vi "pi_control.vi"() -> ()   [LabVIEW 2020]
uses:
  <vilib>/Platform/TimedLoop/XDataNode/timing_clust.ctl
  <vilib>/Platform/TimedLoop/XDataNode/nitl_modes.ctl
  <vilib>/Platform/TimedLoop/XDataNode/wakeup.ctl
  <vilib>/Model Interface Toolkit/Model Interface Toolkit.lvclass/Model Interface Toolkit.ctl
  <vilib>/Model Interface Toolkit/Model Update.vi
  <vilib>/Model Interface Toolkit/Tick Model.vi
  <vilib>/Model Interface Toolkit/Probe Signals.vi
  <vilib>/Model Interface Toolkit/Multirate/Dispatch Model Tasks.vi
  <vilib>/Model Interface Toolkit/Call Model Start Routine.vi
  <vilib>/Model Interface Toolkit/Handle Error.vi
  <vilib>/Model Interface Toolkit/Multirate/Wait on Tasks.vi
  <vilib>/Model Interface Toolkit/Get Inport Paths.vi
  <vilib>/Model Interface Toolkit/Get Outport Paths.vi
  <vilib>/Model Interface Toolkit/Check Error.vi
  <vilib>/Model Interface Toolkit/Generate Error Cluster.vi
  <vilib>/Platform/TimedLoop/scheduler/LVUserAPI/Fire Software-Triggered Timing Source.vi
  <vilib>/Platform/TimedLoop/XDataNode/XDataNode.xnode
  <vilib>/Model Interface Toolkit/Model Interface Toolkit.lvclass
  <vilib>/Platform/TimedLoop/XDataNode/XDNodeRunTimeDep.lvlib
panel:
  in  "选项卡控件":enum32{"参数配置", "控制器及车辆状态评估"}(tab)
  out "Inports":string[](array[string])
  out "Outports":string[](array[string])
  in  "Model Path":path=path "C:/ni-rt/NIVeriStand2010/Models/TSMC_V2.dll"
  in  "数据储存路径":path=path "C:/ni-rt/startup/data/test5.tdms"
  out "controler output data":dbl[](array[numeric])
  out "CarSim Output Data":dbl[](array[numeric]) format="%.2f"
  out "Time Step":dbl=0.001 format="%.4f"
  out "Current Time":dbl format="%.2f"
  out "Start Time":dbl format="%.2f"
  out "Stop Time":dbl=0.001 format="%.4f"
  out "Overrun":i32
  out "x*y":dbl
  out "相平面图":cluster{"X":dbl, "Y":dbl}[](graph)
  out "瞬态误差":cluster{"下界":dbl, "误差":dbl, "上界":dbl}(graph)
  out "波形图表":T1(graph)
  in  "stop":bool
  # "Simulation"
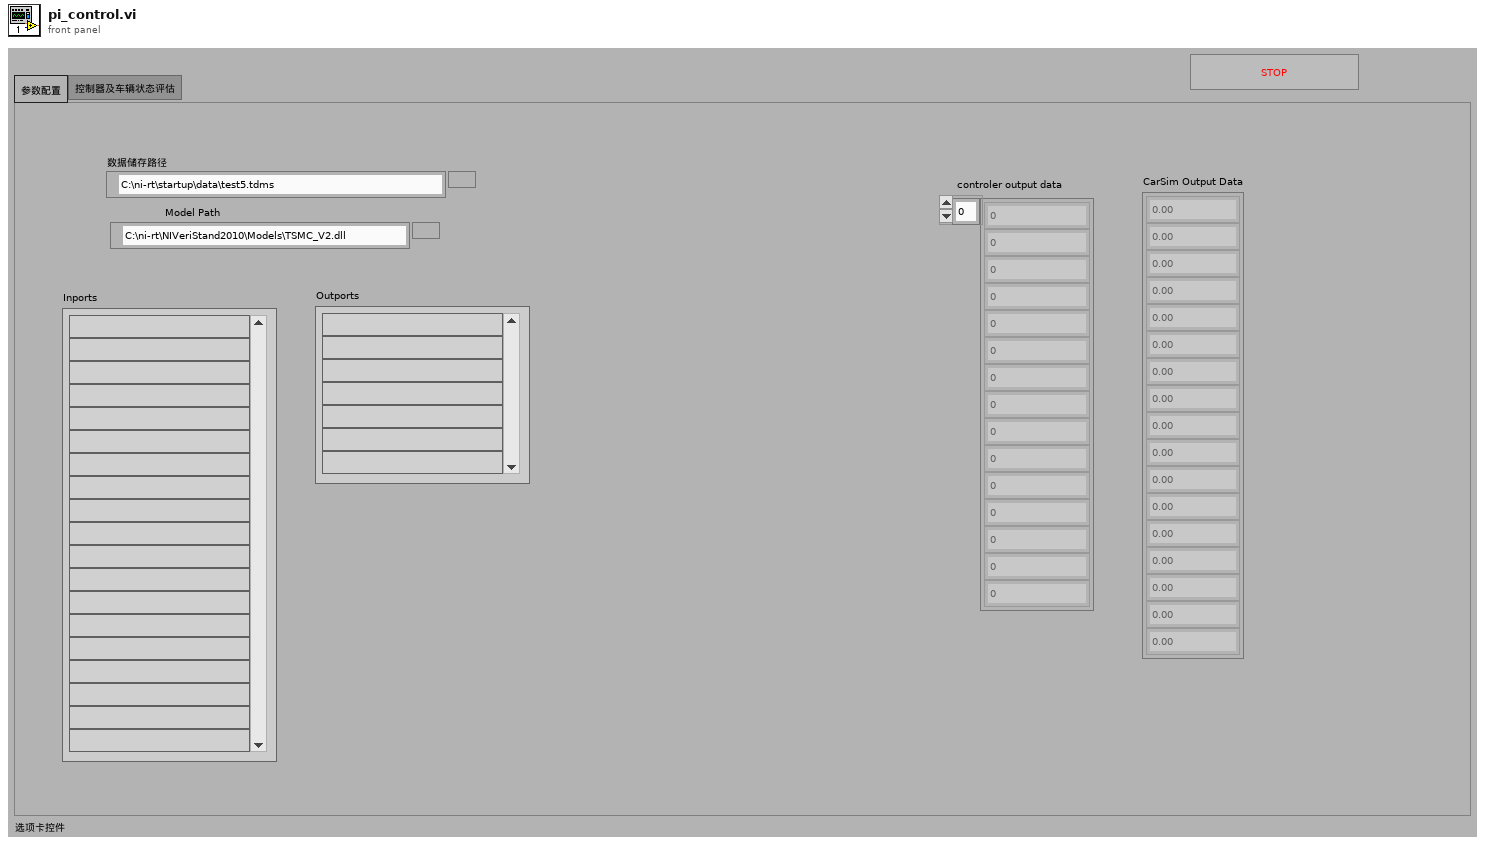
[diagram p1: front panel]
types:
  T1 = cluster{"[0]":dbl, "[1]":dbl, "[2]":dbl, "[3]":dbl, "[4]":dbl}
  T2 = enum16{"open", "open or create", "create or replace", "create", "open (read-only)"}
  T3 = typedef "XDNodeRunTimeDep.lvlib/timing_clust.ctl" = cluster{"Expected End [f-1]":u64, "Actual End [f-1]":u64, "Finished Late? [f-1]":bool, "Expected End [i-1]":u64, "Actual End [i-1]":u64, "Finished Late? [i-1]":bool, "Expected Start [i]":u64, "Actual Start [i]":u64, "Expected Start [f]":u64, "Actual Start [f]":u64, "Source Name":string, "Structure Name":string, "Period":i64, "Deadline":i64, "Offset":i64, "Start":i64, "Priority":i32, "Timeout":i32, "Mode":T4, "Wakeup Reason":T5, "Error":errorcluster, "Source Type":string, "Secondary Source Type":string, "Global End Time":u64, "Global Start Time":u64, "Frame Duration":u64, "Iteration Duration":u64, "Assigned CPU":i32, "I/O Scan Engine Mode":u32}
  T4 = typedef "XDNodeRunTimeDep.lvlib/nitl_modes.ctl" = enum32{"No Change", "Process missed periods, maintain original phase", "Discard missed periods, maintain original phase", "Process missed periods, ignore original phase", "Discard missed periods, ignore original phase"}
  T5 = typedef "XDNodeRunTimeDep.lvlib/wakeup.ctl" = enum32{"Normal", "Aborted", "Asynchronous wakeup", "Timing source error", "Timed loop error", "Timeout"}
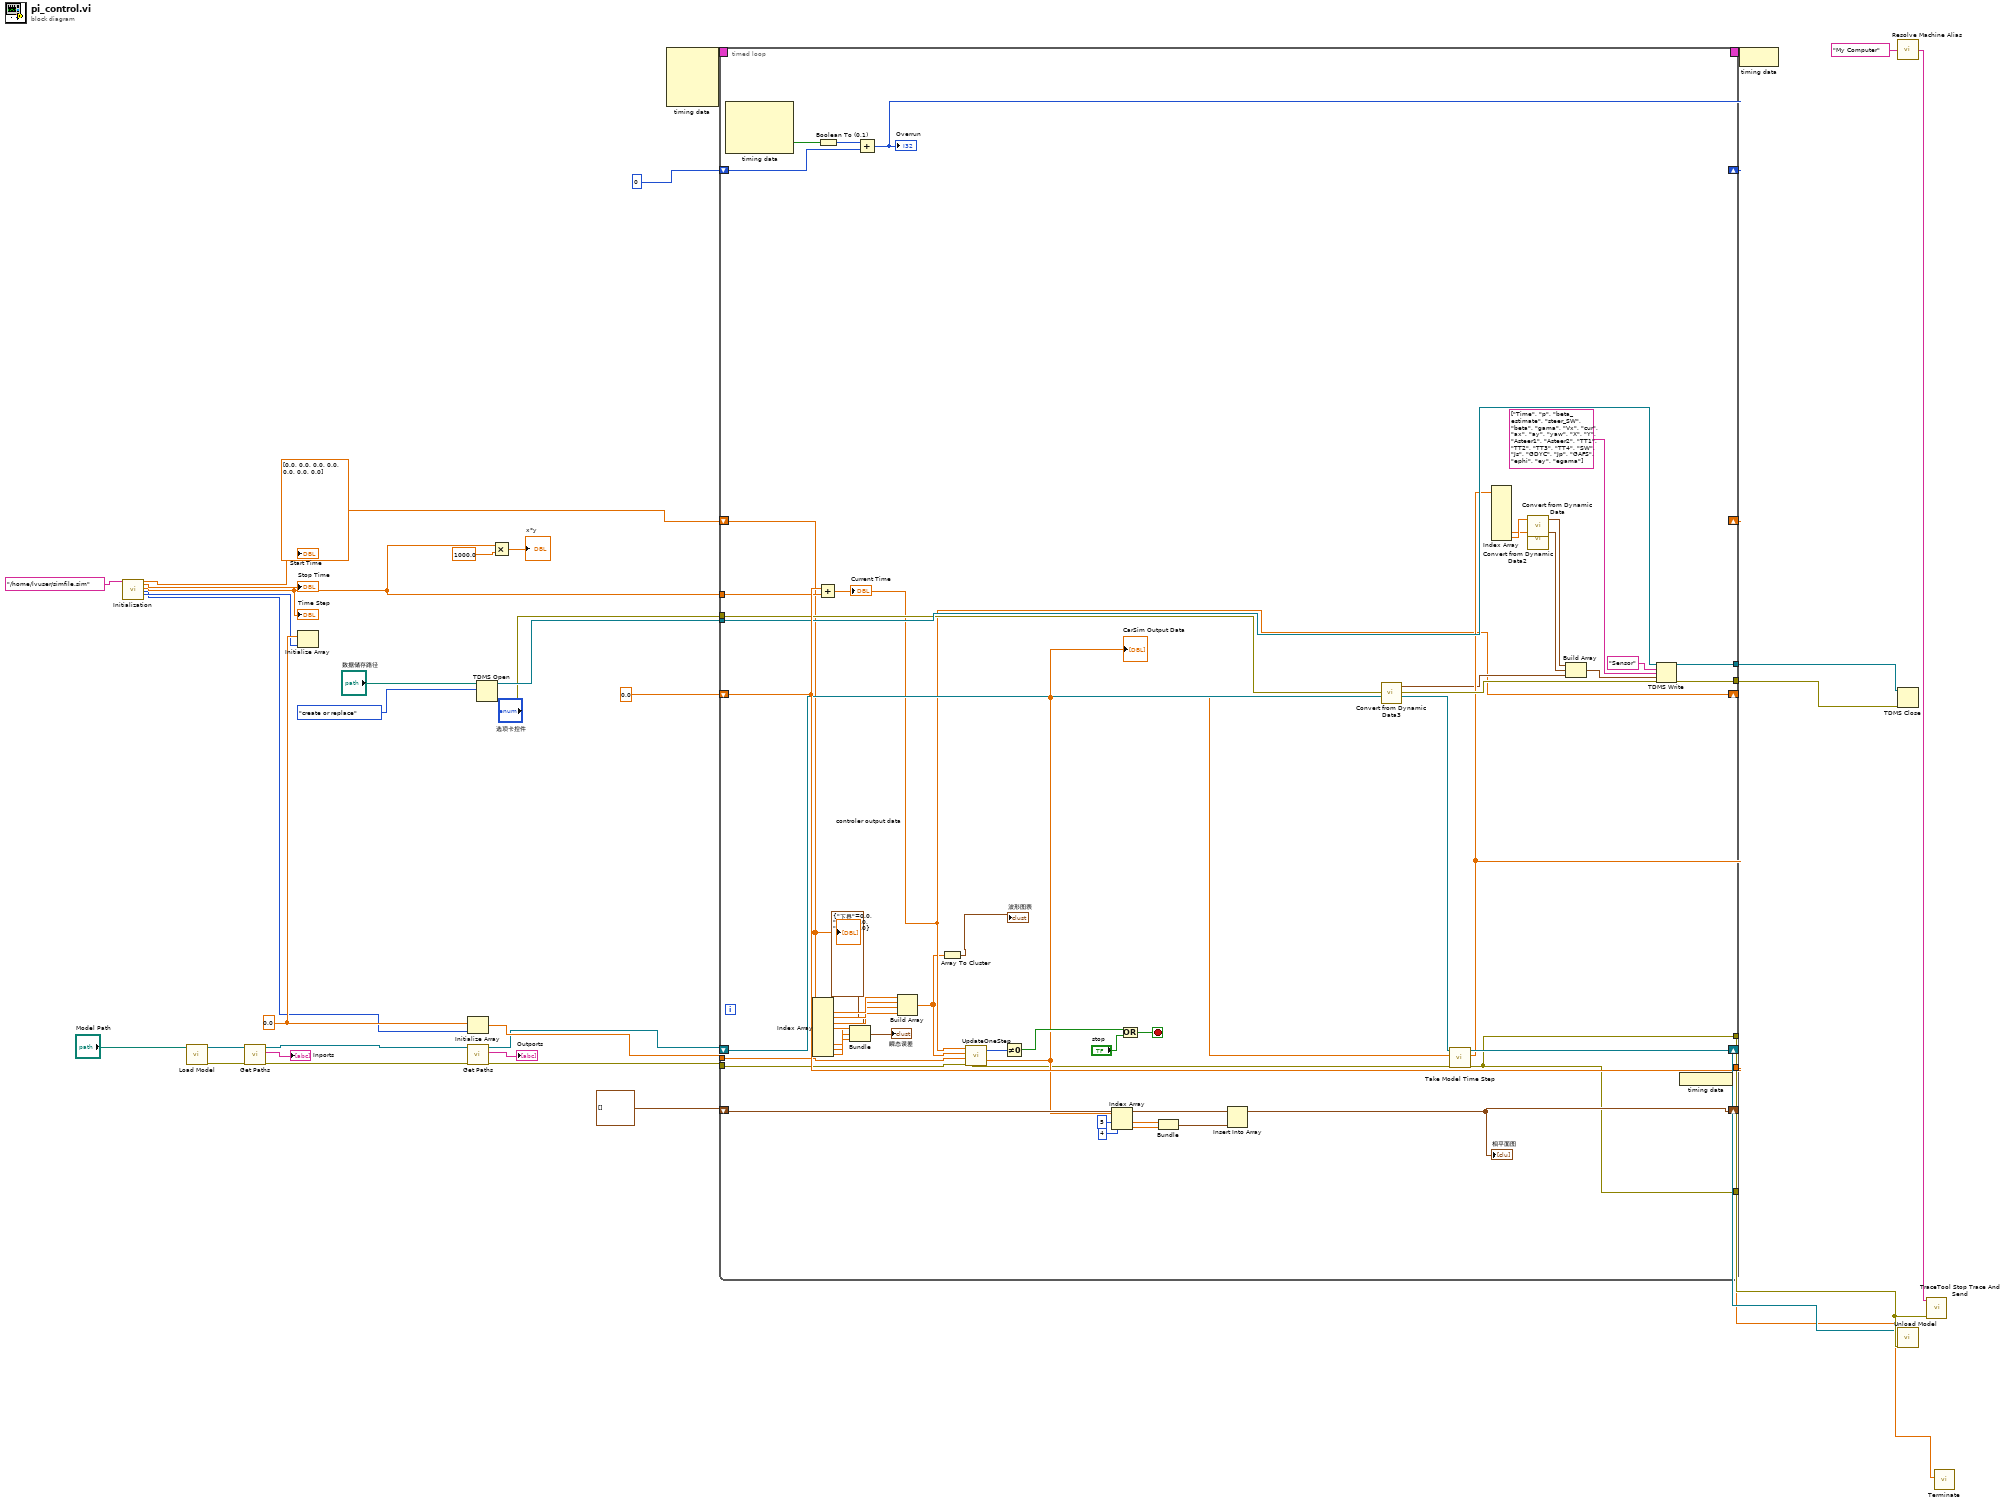
[diagram p0: block diagram]
diagram:
  w34 = 0.0
  n1 = call "Initialization.vi"("Simfile"="/home/lvuser/simfile.sim") -> ("Start Time"=→"Start Time":dbl, "Stop Time"=→"Stop Time":dbl, "Time Step"=w4:dbl, "Number Input"=w3:i16, "Number Output"=w2:i16)  [unwired: 13 in, 1 out]
  "Time Step" <- w4
  n2 = call <vilib>:"Load Model.vi"("Model Path"="Model Path") -> ("error out"=w22:errorcluster, "Model out"=w23:refnum<class "Model Interface Toolkit.lvclass">)  [unwired: 9 in]
  n3 = call-poly <vilib>:"Get Paths.vi"("error in (no error)"=w22, "Model in"=w23) -> ("error out"=w27:errorcluster, "Inport Paths"=→"Inports":string[], "Model out"=w26:refnum<class "Model Interface Toolkit.lvclass">)  [unwired: 7 in]
  n4 = Initialize Array ("初始化数组")(w34, w3) -> ()  [unwired: 1 out]
  n5 = Initialize Array ("初始化数组")(w34, w2) -> (w33:dbl[])
  n6 = call-poly <vilib>:"Get Paths.vi"("error in (no error)"=w27, "Model in"=w26) -> ("error out"=w20:errorcluster, "Outport Paths"=→"Outports":string[], "Model out"=w21:refnum<class "Model Interface Toolkit.lvclass">)  [unwired: 7 in]
  n7 = TDMS Open ("TDMS打开")(10:T2."create or replace" ("operation (0:open)"), 11:"数据储存路径") -> (0:w11:errorcluster, 3:w12:refnum<k34>)  [unwired: 5 in]
  n8 = Multiply ("乘")(x=w4, y=1000.0) -> (x*y=→"x*y":dbl)
  n9 = node-c288() -> (w36:T3)  [unwired: 4 in]
  n10 = timed-loop "定时循环" {
    timing: w36 -> [_]
    timing-out: [_] -> w35
    tunnel: w33 -> [w41]
    tunnel: w4 -> [w82]
    shift-right: [w43] -> _
    shift-left: 0.0 -> [w83]
    tunnel: [w83] -> w7
    shift-right: [w79] -> _
    shift-left: 0 -> [w80]
    tunnel: [w44] -> w19
    tunnel: w20 -> [w40]
    shift-right: [w67] -> _
    shift-left: dbl[] [0.0, 0.0, 0.0, 0.0, 0.0, 0.0, 0.0] ("Outport Array out") -> [w66]
    shift-right: [w76] -> w16
    shift-left: w21 -> [w77]
    tunnel: w12 -> [w75]
    tunnel: w11 -> [w74]
    tunnel: [w71] -> w10
    tunnel: [w70] -> w9
    shift-right: [w53] -> _
    shift-left: cluster{dbl, dbl}[] [] -> [w57]
    tunnel: [w44] -> _
    stop <- w85 stop-if-true
    n11 = node-c288() -> (w78:bool)  [unwired: 1 in, 3 out]
    n12 = Index Array(array=w66) -> (element #1=w61:dbl, element #2=w60:dbl, element #3=w59:dbl, element #4=w58:dbl, element #7=w45:dbl, element #8=w46:dbl, element #9=w47:dbl)  [unwired: 9 in, 2 out]
    n13 = Boolean To (0,1) ("布尔值至(0,1)转换")(Boolean=w78) -> (0, 1=w81:i16)
    n14 = Add ("加")(x=w83, y=w82) -> (x+y=w43:dbl)
    "Current Time" <- w43
    n15 = Bundle(cluster=cluster{"下界":dbl, "误差":dbl, "上界":dbl} {"下界"=0.0, "误差"=0.0, "上界"=0.0} ("簇"), "下界"=w45, "误差"=w46, "上界"=w47) -> (→"瞬态误差":cluster{"下界":dbl, "误差":dbl, "上界":dbl})
    n16 = Add ("加")(x=w81, y=w80) -> (x+y=w79:i32)
    "Overrun" <- w79
    n17 = Build Array ("创建数组")(w61, w60, w59, w58) -> (w42:dbl[])
    n18 = Array To Cluster ("数组至簇转换")(array=w42) -> (cluster=→"波形图表":T1)
    n19 = call "UpdateOneStep.vi"("error in (no error)"=w40, "init output"=w41, "input data"=w42, "time"=w43) -> ("error out"=w37:errorcluster, "output data"=w38:dbl[], "Func Return"=w39:i16)  [unwired: 5 in]
    "CarSim Output Data" <- w38
    n20 = Not Equal To 0? ("不等于0？")(x=w39) -> (x != 0?=w86:bool)
    n21 = Index Array(array=w38, index #1=5 ("索引"), index #2=4 ("索引")) -> (element #1=w55:dbl, element #2=w54:dbl)
    n22 = Or ("或")(x=w86, y="stop") -> (x .or. y?=w85:bool)
    n23 = Bundle(w55, w54) -> (w56:cluster{dbl, dbl})  [unwired: 1 in]
    n24 = Insert Into Array(array=w57, new element=w56) -> (w53:cluster{dbl, dbl}[])  [unwired: 1 in]
    "相平面图" <- w53
    n25 = call "Convert from Dynamic Data3"() -> ("Waveform"=w62:waveform(dbl))  [unwired: 4 in]
    n26 = call <vilib>:"Take Model Time Step.vi"("error in (no error)"=w37, "Inport Array"=w38, "Model in"=w77) -> ("error out"=w44:errorcluster, "Outport Array out"=w67:dbl[], "Model out"=w76:refnum<class "Model Interface Toolkit.lvclass">)  [unwired: 6 in]
    n27 = Index Array ("索引数组")(array=w67) -> (element #7=w63:dbl, element #8=w65:dbl)  [unwired: 8 in, 6 out]
    n28 = call "Convert from Dynamic Data"("Dynamic Data Type"=w65) -> ("Waveform"=w69:waveform(dbl))  [unwired: 3 in]
    n29 = call "Convert from Dynamic Data2"("Dynamic Data Type"=w63) -> ("Waveform"=w64:waveform(dbl))  [unwired: 3 in]
    n30 = Build Array ("创建数组")(w69, w64, w62) -> (w68:waveform(dbl)[])
    n31 = TDMS Write ("TDMS写入")(0:w75, 5:"Sensor" ("group name in (Untitled)"), 7:string[] ["Time", "p", "beta_estimate", "steer_SW", "beta", "gama", "Vx", "cur", "ax", "ay", "yaw", "X", "Y", "Asteer1", "Asteer2", "TT1", "TT2", "TT3", "TT4", "SW", "Js", "GDYC", "Jp", "GAFS", "ephi", "ey", "egama"] ("channel name(s) in (Untitled)"), 9:w68, 11:w74) -> (4:w71:refnum<k34>, 15:w70:errorcluster)  [unwired: 1 in, 2 out]
    n32 = node-c288() -> ()  [unwired: 1 out]
    "controler output data" <- w66
  }
  n33 = node-c288(w35) -> ()
  n34 = call <vilib>:"Resolve Machine Alias.vi"("Machine Alias"="My Computer" ("Trace Host Network Address")) -> ("Network Identity"=w30:string)  [unwired: 2 in, 2 out]
  n35 = TDMS Close ("TDMS关闭")(8:w9, 11:w10) -> ()  [unwired: 2 out]
  n36 = call <vilib>:"Unload Model.vi"("error in (no error)"=w19, "Model in"=w16) -> ()  [unwired: 9 in, 1 out]
  n37 = call <vilib>:"TraceTool Stop Trace And Send.vi"("error in (no error)"=w19, "Trace Host Network Address"=w30) -> ()  [unwired: 9 in, 1 out]
  n38 = call "Terminate.vi"("time"=w7) -> ()  [unwired: 10 in, 1 out]
